vi "LinearSystemLoop_SngJntArm_Execute.vi"(5 "LinearSystem_ID_SngJntArm_Model":T2={"DCMOTOR_TYPES"=enum."NEO", "Num Motors"=1, "ArmLength_M"=0.75, "massKg"=26.0, "Gearing"=128.0, "MOI kgm2"=26.0, "Estimate MOI"=TRUE} {"MOI kgm2" format="%#_13g"; "Gearing" format="%#_13g"; "massKg" format="%#_13g"; "ArmLength_M" format="%#_13g"}, 6 "dT Sec":dbl=0.02, 7 "LinearSystem_SngJntArm_Ctrl_Params":T1={"Ang Model Std Dev Rad"=0.5, "Ang Meas Std Dev Rad"=0.02, "Ang Ctrl Tol Rad"=0.06, "Max Ctrl Out V"=12.0, "Vel Model Std Dev Rad/Sec"=20.0, "Vel Ctrl Tol Rad/Sec"=0.8}, 9 "Process Variable\nRadians":dbl, 10 "Ang Vel SP Rad":dbl format="%#_13g", 11 "Ang Pos SP Rad":dbl) -> (0 "Error":bool, 1 "Filtered Vel Rad/Sec":dbl, 2 "Filtered Angle Radians":dbl, 3 "Motor Dmd":dbl, 4 "out Linear System Loop":T4)   [LabVIEW 2019, in "Trajectory_Library.lvlib"]
doc: "Model and control a single jointed arm system using a Kalman FIlter and LQR controller. This is a single call LabVIEW function.\n\nThe single jointed arm linear system definition is:\n - States\n - angle position (Rad)\n - velocity (Rad/Sec)\n - Inputs:\n - motor voltage\n - Outputs:\n - angle position (rad)\n\n\nInputs:\n - LinearSystemId SngJntArm Model -- cluster -- Packed parameters used to create Single Jointed Arm linear system.\n - LineaarSystem SngJntArm Ctrl -- cluster -- Packed parameters used by Kalman Filter and LQR to control the system.\n - Ang Pos Setpoint -- double -- Desired arm angle (radians)\n - Ang Vel Setpiont -- double -- Desired arm speed setpoint (Rad/sec, Default: 0)\n - PV -- double -- Measured arm angle (radians)\n - dT -- double -- Update time (Seconds, Default: 0.02)\n\nOutputs:\n - Motor Dmd - double -- Motor demand (+/- 1.0)\n - Kalman FIltered angle -- double -- Filtered angle (radians)\n - Kalman filtered velocity -- double -- Filtered velocity (Rad/Sec)\n - Error -- boolean -- If TRUE an error occured."
uses:
  Trajectory_Library.lvlib
  <vilib>/Analysis/Matrix/Datatypes/RealMatrix.ctl
  <vilib>/Analysis/Matrix/NI_Matrix.lvlib
  TypeDef/LINEAR_QUADRATIC_REGULATOR.ctl
  TypeDef/LINEAR_PLANT_INV_FF.ctl
  TypeDef/LINEAR_SYSTEM.ctl
  TypeDef/KALMAN_FILTER.ctl
  TypeDef/LINEAR_SYSTEM_LOOP.ctl
  Enum/DCMOTOR_TYPES_ENUM.ctl
  TypeDef/LINEAR_SYSTEM_ID_SINGLE_JOINT_ARM_MODEL.ctl
  TypeDef/LINEAR_SYSTEM_LOOP_SNGJNTARM_CTRL_PARAMS.ctl
panel:
  # "<States,1>"
  # "<FUTURE --- CLAMP TYPE -- For now\nuse Normalize>"
  # "Steady State Gain  \n<States,Outputs>"
  # "State Estimate <Statess,1>"
  # "<States,States>"
  # "<States,Inputs>"
  # "<Outputs,States>"
  # "<Outputs,Inputs>"
  # "<States,1>"
  # "<Inputs,1>"
  # "<States,Inputs>"
  # "<States,States>"
  # "Ref State <States,1>"
  # "Comp and capped \noutput <Inputs,1>"
  # "Controller gain\n<Inputs,States>"
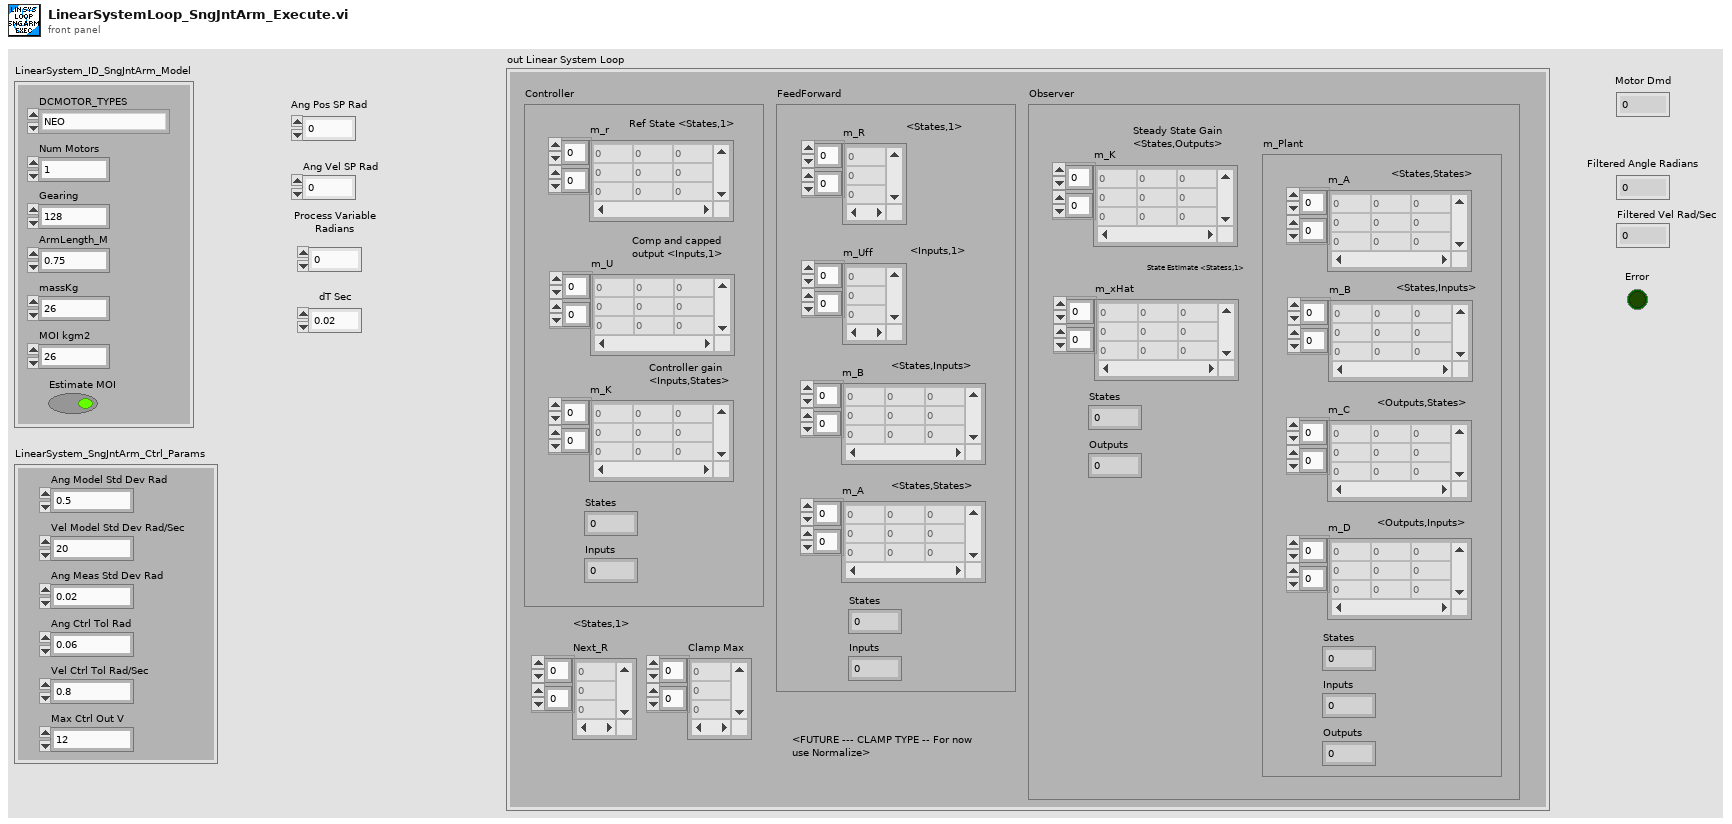
[diagram p1: front panel]
types:
  T1 = typedef "Trajectory_Library.lvlib/LINEAR_SYSTEM_LOOP_SNGJNTARM_CTRL_PARAMS.ctl" = cluster{"Ang Model Std Dev Rad":dbl, "Ang Meas Std Dev Rad":dbl, "Ang Ctrl Tol Rad":dbl, "Max Ctrl Out V":dbl, "Vel Model Std Dev Rad/Sec":dbl, "Vel Ctrl Tol Rad/Sec":dbl}
  T2 = typedef "Trajectory_Library.lvlib/LINEAR_SYSTEM_ID_SINGLE_JOINT_ARM_MODEL.ctl" = cluster{"DCMOTOR_TYPES":T3, "Num Motors":i32, "ArmLength_M":dbl, "massKg":dbl, "Gearing":dbl, "MOI kgm2":dbl, "Estimate MOI":bool}
  T3 = typedef "Trajectory_Library.lvlib/DCMOTOR_TYPES_ENUM.ctl" = enum16{"CIM", "AndyMark 9015", "Andy Mark RS 775 125", "Bag", "BaneBots RS 550", "BaneBots RS 775", "Falcon 500", "Mini CIM", "NEO", "NEO 550", "Romi BuiltIn", "Vex 775 Pro", "Snow Blower AM 2235A", "Bosch Seat AM 3493", "Falcon 500 FOC", "Kraken X60", "Kraken X60 FOC", "NEO Vortex"}
  T4 = typedef "Trajectory_Library.lvlib/LINEAR_SYSTEM_LOOP.ctl" = cluster{"Controller":T5, "FeedForward":T7, "Observer":T8, "Next_R":T6, "Clamp Max":T6}
  T5 = typedef "Trajectory_Library.lvlib/LINEAR_QUADRATIC_REGULATOR.ctl" = cluster{"m_r":T6, "m_U":T6, "m_K":T6, "States":i32, "Inputs":i32}
  T6 = typedef "NI_Matrix.lvlib/RealMatrix.ctl" = dbl[][]
  T7 = typedef "Trajectory_Library.lvlib/LINEAR_PLANT_INV_FF.ctl" = cluster{"m_R":T6, "m_Uff":T6, "m_B":T6, "m_A":T6, "States":i32, "Inputs":i32}
  T8 = typedef "Trajectory_Library.lvlib/KALMAN_FILTER.ctl" = cluster{"m_K":T6, "m_xHat":T6, "States":i32, "Outputs":i32, "m_Plant":T9}
  T9 = typedef "Trajectory_Library.lvlib/LINEAR_SYSTEM.ctl" = cluster{"m_A":T6, "m_B":T6, "m_C":T6, "m_D":T6, "States":i32, "Inputs":i32, "Outputs":i32}
  T10 = typedef "Trajectory_Library.lvlib/DCMOTOR.CTL" = cluster{"nominalVoltage_Volts":dbl, "StallTorque_NM":dbl, "StallCurrent_Amps":dbl, "FreeCurrent_Amps":dbl, "FreeSpeed_RadPerSec":dbl, "R_Ohms":dbl, "KvINV_RadPerSecPerVolt":dbl, "Kt_NMPerAmp":dbl, "L_H":dbl, "Jr_KgM2":dbl}
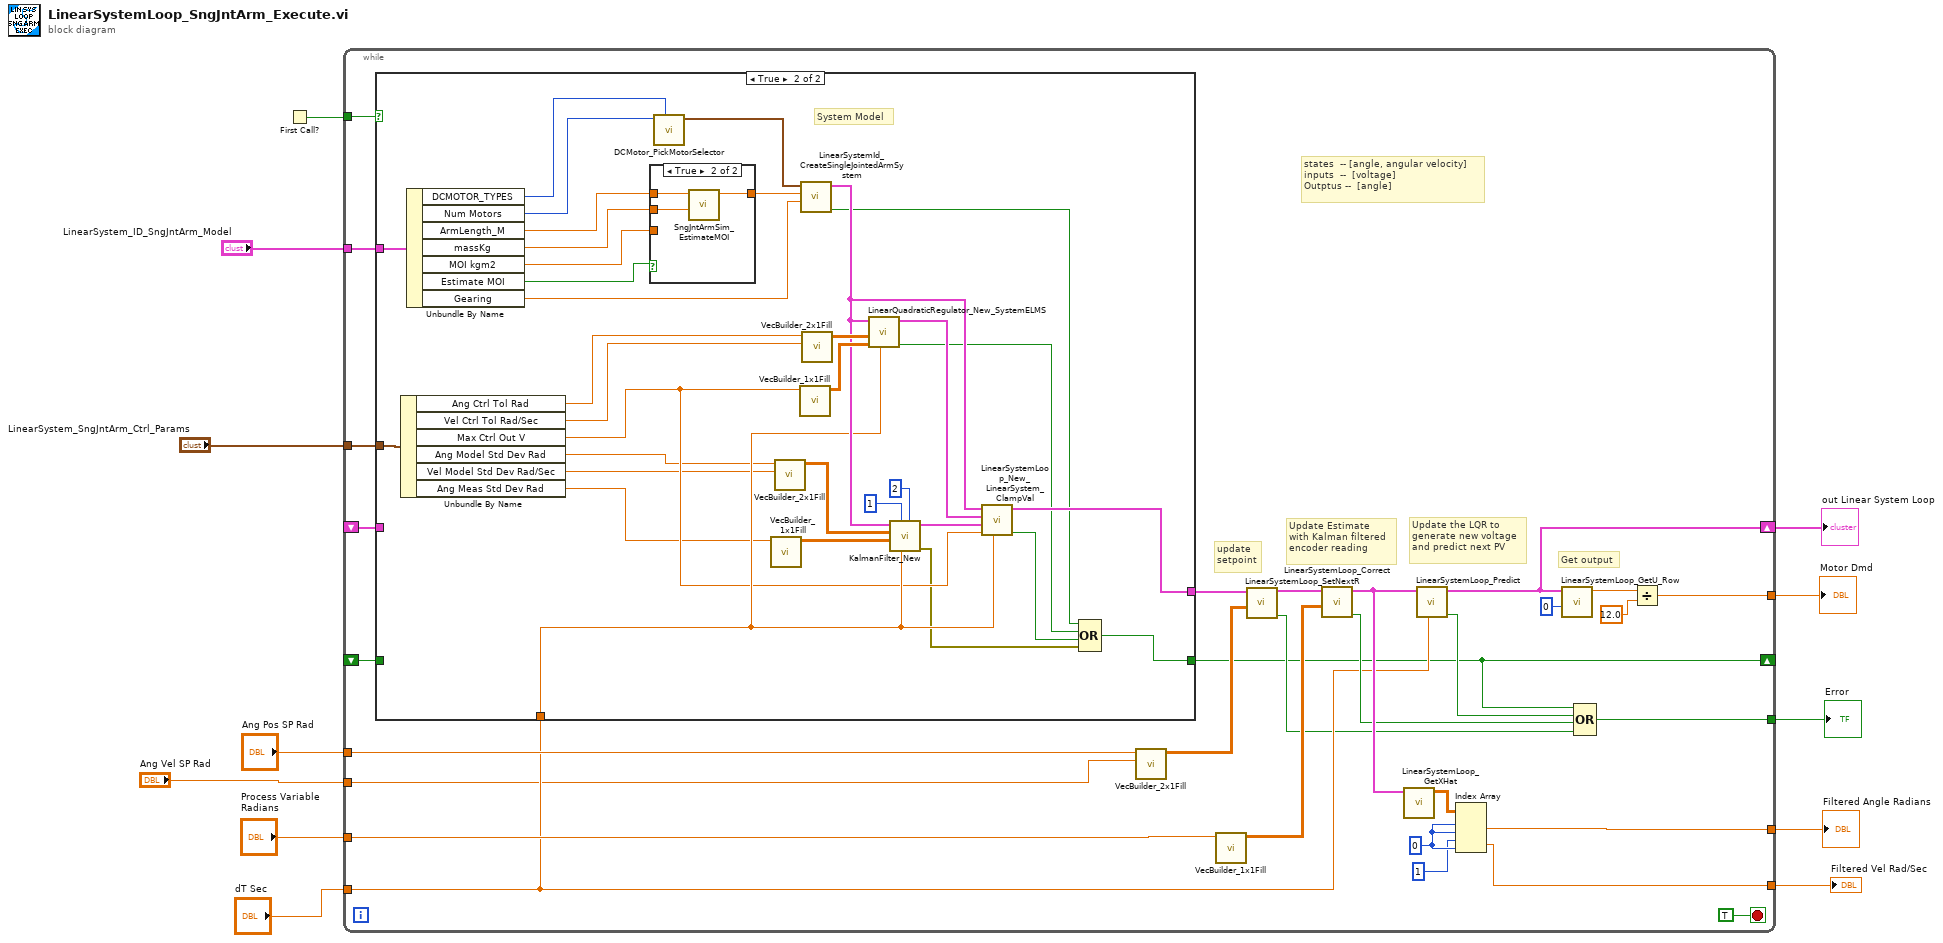
[diagram p0: block diagram]
diagram:
  n1 = First Call?() -> (First Call?: T/F=w4:bool)
  n2 = while {
    tunnel: "Ang Pos SP Rad" -> [w42]
    tunnel: "Process Variable\nRadians" -> [w40]
    tunnel: [w35] -> w9
    tunnel: [w30] -> w8
    tunnel: [w27] -> w7
    tunnel: "dT Sec" -> [w24]
    tunnel: "LinearSystem_ID_SngJntArm_Model" -> [w25]
    shift-right: [w38] -> w10
    shift-left: _ -> [w22]
    tunnel: w4 -> [w21]
    tunnel: "Ang Vel SP Rad" -> [w20]
    tunnel: "LinearSystem_SngJntArm_Ctrl_Params" -> [w19]
    shift-right: [w17] -> _
    shift-left: _ -> [w16]
    tunnel: [w13] -> w1
    stop <- TRUE stop-if-true
    w15 = 0 ("index (row)")
    # "states  -- [angle, angular velocity] \ninputs  --  [voltage]\nOutptus --  [angle]"
    # "Get output"
    # "Update the LQR to \ngenerate new voltage\nand predict next PV"
    # "update \nsetpoint"
    # "Update Estimate\nwith Kalman filtered\nencoder reading"
    n3 = case shown="True" w21 {
      tunnel: w25 -> [_ w75]
      tunnel: w24 -> [_ w57]
      tunnel: [w44 w58] -> w23
      tunnel: w22 -> [w44 _]
      tunnel: w19 -> [_ w56]
      tunnel: [w43 w45] -> w17
      tunnel: w16 -> [w43 _]
      frame False {
      }
      frame True {
        # "System Model"
        n4 = Unbundle By Name(w56) -> ("Ang Ctrl Tol Rad"=w55:dbl, "Vel Ctrl Tol Rad/Sec"=w54:dbl, "Max Ctrl Out V"=w53:dbl, "Ang Model Std Dev Rad"=w52:dbl, "Vel Model Std Dev Rad/Sec"=w51:dbl, "Ang Meas Std Dev Rad"=w50:dbl)
        n5 = Unbundle By Name(w75) -> ("DCMOTOR_TYPES"=w69:T3, "Num Motors"=w68:i32, "ArmLength_M"=w74:dbl, "massKg"=w73:dbl, "MOI kgm2"=w71:dbl, "Estimate MOI"=w72:bool, "Gearing"=w70:dbl)
        n6 = case shown="True" w72 {
          tunnel: [w78 w81] -> w77
          tunnel: w74 -> [_ w80]
          tunnel: w73 -> [_ w79]
          tunnel: w71 -> [w78 _]
          frame False {
          }
          frame True {
            n7 = call "SngJntArmSim_EstimateMOI.vi"("ArmMass_Kg"=w79, "ArmLength_M"=w80) -> ("MOI"=w81:dbl)  [unwired: 9 in]
          }
        }
        n8 = call "DCMotor_PickMotorSelector.vi"("DCMOTOR_TYPES"=w69, "Num Motors"=w68) -> ("DCMOTOR"=w76:T10)  [unwired: 9 in]
        n9 = call "VecBuilder_1x1Fill.vi"("R0_C0"=w50) -> ("output matrix"=w67:T6)  [unwired: 10 in]
        n10 = call "VecBuilder_2x1Fill.vi"("R1"=w51, "R0"=w52) -> ("output matrix"=w66:T6)  [unwired: 9 in]
        n11 = call "VecBuilder_1x1Fill.vi"("R0_C0"=w53) -> ("output matrix"=w64:T6)  [unwired: 10 in]
        n12 = call "LinearSystemId_CreateSingleJointedArmSystem.vi"("G"=w70, "jKgSquaredMeters"=w77, "DCMOTOR"=w76) -> ("Size Coerced"=w49:bool, "Linearsystem"=w62:T9)  [unwired: 7 in]
        n13 = call "VecBuilder_2x1Fill.vi"("R1"=w54, "R0"=w55) -> ("output matrix"=w63:T6)  [unwired: 9 in]
        n14 = call "LinearQuadraticRegulator_New_SystemELMS.vi"("dt_Seconds"=w57, "Relms"=w64, "Qelms"=w63, "LINEARSYSTEM"=w62) -> ("Error"=w48:bool, "LinearQuadraticRegulator"=w61:T5)  [unwired: 6 in]
        n15 = call "KalmanFilter_New.vi"("States"=2, "dt_Seconds"=w57, "Outputs"=1, "MeasurementStdDevs"=w67, "StateStdDevs"=w66, "Plant"=w62) -> ("Error"=w46:errorcluster, "KalmanFilter"=w59:T8)  [unwired: 4 in]
        n16 = call "LinearSystemLoop_New_LinearSystem_ClampVal.vi"("dT_Seconds"=w57, "Max_Voltage"=w53, "Observer"=w59, "Controller"=w61, "Plant"=w62) -> ("Error"=w47:bool, "Linear System Loop"=w58:T4)  [unwired: 5 in]
        n17 = Compound Arithmetic op=OR(w49, w48, w47, w46) -> (w45:bool)
      }
    }
    n18 = call "VecBuilder_2x1Fill.vi"("R1"=w20, "R0"=w42) -> ("output matrix"=w41:T6)  [unwired: 9 in]
    n19 = call "VecBuilder_1x1Fill.vi"("R0_C0"=w40) -> ("output matrix"=w33:T6)  [unwired: 10 in]
    n20 = call "LinearSystemLoop_SetNextR.vi"("R"=w41, "input inear System Loop"=w23) -> ("Size Coerced"=w18:bool, "out Linear System Loop"=w39:T4)  [unwired: 8 in]
    n21 = call "LinearSystemLoop_Correct.vi"("Y"=w33, "input inear System Loop"=w39) -> ("Error"=w31:bool, "out Linear System Loop"=w36:T4)  [unwired: 8 in]
    n22 = call "LinearSystemLoop_GetXHat.vi"("input inear System Loop"=w36) -> ("XHat"=w34:T6)  [unwired: 10 in]
    n23 = call "LinearSystemLoop_Predict.vi"("dT_Seconds"=w24, "input inear System Loop"=w36) -> ("Error"=w32:bool, "out Linear System Loop"=w38:T4)  [unwired: 8 in]
    n24 = Index Array(array=w34, index (row) #1=w15, index (col) #1=w15, index (row) #2=1 ("index (row)"), index (col) #2=w15) -> (element #1=w35:dbl, element #2=w13:dbl)
    n25 = call "LinearSystemLoop_GetU_Row.vi"("Row"=0, "input inear System Loop"=w38) -> ("U"=w29:dbl)  [unwired: 9 in]
    n26 = Compound Arithmetic op=OR(w17, w32, w31, w18) -> (w30:bool)
    n27 = Divide(x=w29, y=12.0) -> (x/y=w27:dbl)
  }
  "Motor Dmd" <- w7
  "out Linear System Loop" <- w10
  "Filtered Angle Radians" <- w9
  "Error" <- w8
  "Filtered Vel Rad/Sec" <- w1
